vi "Test Configuration Flatten.vi"() -> ()   [LabVIEW 2021]
uses:
  PCAP_Universal/Typedef/Buffer Configuration Data.ctl
  PCAP_Universal/CIF_Iceoryx_PCAP_Universal.lvclass
panel:
  out "Pass":bool
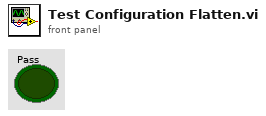
[diagram p1: front panel]
types:
  T1 = typedef "CIF_Iceoryx_PCAP_Universal.lvclass/Buffer Configuration Data.ctl" = cluster{"Backpressure":bool}
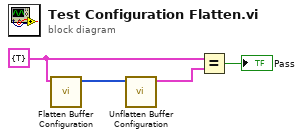
[diagram p0: block diagram]
diagram:
  w1 = T1 {"Backpressure"=TRUE} ("Buffer Configuration")
  n1 = call "Flatten Buffer Configuration.vi"("Buffer Configuration"=w1) -> ("Flattened Configuration"=w4:u8[])  [unwired: 10 in]
  n2 = call "Unflatten Buffer Configuration.vi"("Flattened Configuration"=w4) -> ("Buffer Configuration"=w3:T1)  [unwired: 10 in]
  n3 = Equal?(x=w1, y=w3) -> (x = y?=→"Pass":bool)
